vi "Own20261012_GetArrayInfo.vi"() -> ()   [LabVIEW 2024]
panel:
  out "error out":errorcluster caption="错误输出"
  out "terminal_id":refnum<vi>
  out "element_id":refnum<vi>
  out "dimensions":u32
  in  "array_id":u32
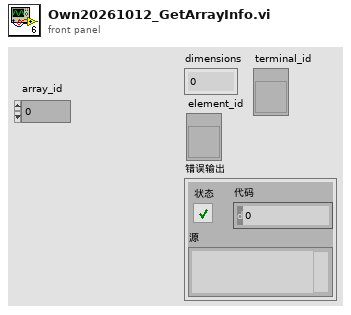
[diagram p1: front panel]
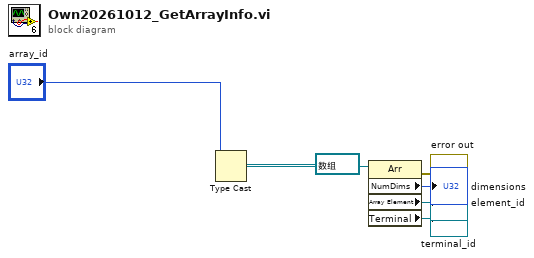
[diagram p0: block diagram]
diagram:
  n1 = Type Cast(type=refnum<vi> refnum ("引用"), x="array_id") -> (*(type *) &x=w5:refnum<vi>)
  n2 = property class="Arr"(reference=w5) -> (error out=→"error out":errorcluster, "NumDims"=→"dimensions":u32, "Array Element"=→"element_id":refnum<vi>, "Terminal"=→"terminal_id":refnum<vi>)  [unwired: 1 in, 1 out]
